vi "Evaluate Bool Group.vi"(8 "error in":errorcluster, 10 "group":cluster{"and_list":string[], "or_list":string[]}, 11 "bool values":cluster{"name":string, "on":bool}[](array[cluster])) -> (0 "error out":errorcluster, 2 "first fail":string, 3 "passes":bool)   [LabVIEW 2026]
doc: "Condition group AND/OR over boolean IO values. Every 'and' name must be found and TRUE; at least one 'or' name must be found and TRUE (an empty 'or' list passes). An empty 'and' list passes. An unknown name fails and is reported as the first failing item."
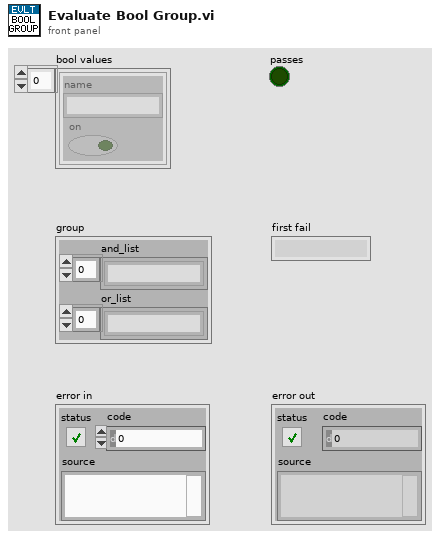
[diagram p1: front panel]
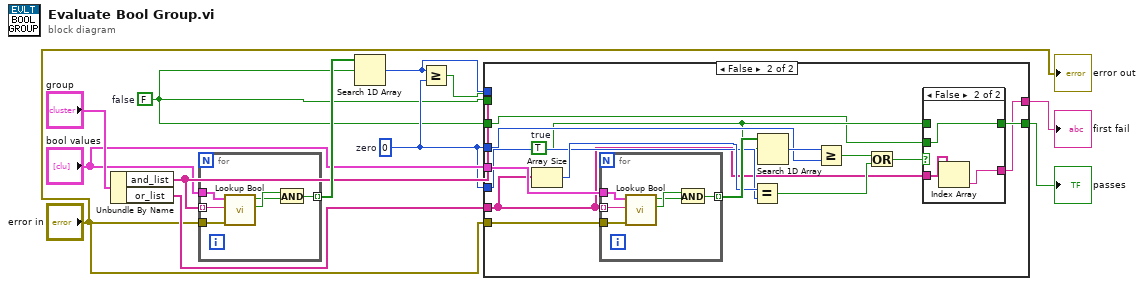
[diagram p0: block diagram]
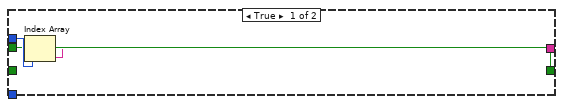
[diagram p2: hidden frame]
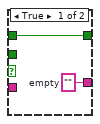
[diagram p3: hidden frame]
diagram:
  w6 = 0  # zero
  w5 = FALSE  # false
  n1 = Unbundle By Name("group") -> ("and_list"=w10:string[], "or_list"=w8:string[])
  n2 = for {
    tunnel: w10 -> [w17] mode=indexing
    tunnel: "bool values" -> [w18]
    tunnel: "error in" -> [w16]
    tunnel: [w13] -> w11 mode=indexing
    n3 = call "Lookup Bool.vi"("error in"=w16, "name"=w17, "bool values"=w18) -> ("found"=w15:bool, "on"=w14:bool)  [unwired: 6 in, 1 out]
    n4 = And(x=w15, y=w14) -> (x .and. y?=w13:bool)
  }
  n5 = Search 1D Array(1D array=w11, element=w5) -> (index of element=w9:i32)  [unwired: 1 in]
  n6 = Greater Or Equal?(x=w9, y=w6) -> (x >= y?=w4:bool)
  n7 = case shown="False" w4 {
    tunnel: w10 -> [w21 _]
    tunnel: w9 -> [w22 _]
    tunnel: w8 -> [_ w28]
    tunnel: [w20 w24] -> w3
    tunnel: w5 -> [w20 _]
    tunnel: [w19 w23] -> w2
    tunnel: "bool values" -> [_ w37]
    tunnel: "error in" -> [_ w36]
    tunnel: w6 -> [_ w33]
    tunnel: w6 -> [_ w31]
    tunnel: w5 -> [_ w26]
    frame True {
      n8 = Index Array(array=w21, index=w22) -> (element=w19:string)
    }
    frame False {
      w27 = TRUE  # true
      n9 = Array Size(array=w28) -> (size(s)=w32:i32)
      n10 = for {
        tunnel: w28 -> [w47] mode=indexing
        tunnel: w37 -> [w48]
        tunnel: w36 -> [w46]
        tunnel: [w43] -> w35 mode=indexing
        n11 = call "Lookup Bool.vi"("error in"=w46, "name"=w47, "bool values"=w48) -> ("found"=w45:bool, "on"=w44:bool)  [unwired: 6 in, 1 out]
        n12 = And(x=w45, y=w44) -> (x .and. y?=w43:bool)
      }
      n13 = Equal?(x=w32, y=w31) -> (x = y?=w29:bool)
      n14 = Search 1D Array(1D array=w35, element=w27) -> (index of element=w34:i32)  [unwired: 1 in]
      n15 = Greater Or Equal?(x=w34, y=w33) -> (x >= y?=w30:bool)
      n16 = Or(x=w30, y=w29) -> (x .or. y?=w25:bool)
      n17 = case shown="False" w25 {
        tunnel: w28 -> [_ w42]
        tunnel: [w39 w41] -> w24
        tunnel: w27 -> [w39 _]
        tunnel: [w38 w40] -> w23
        tunnel: w26 -> [_ w41]
        frame True {
          w38 = ""  # empty
        }
        frame False {
          n18 = Index Array(array=w42) -> (element=w40:string)  [unwired: 1 in]
        }
      }
    }
  }
  "passes" <- w3
  "first fail" <- w2
  "error out" <- "error in"
